vi "ASDE Signal Data Table For New_MS.vi"(4 "S Anal":T4, 6 "F ex Info":T3, 7 "S Table Z":T1, 8 "error in":errorcluster caption="エラー入力", 9 "S Table C2":T2={"R BL (pA)"=0.0, "R STD (pA)"=0.0, "U thre (pA)"=0.0, "D thre (pA)"=0.0, "U thre (n)"=0.0, "D thre (n)"=0.0, "STD smooth Point "=10, "MAX Duration time(s)"=0.01} {"MAX Duration time(s)" format="%#_13g"}, 10 "S Table C1":T6, 11 "S Table C0":T5) -> (0 "error out":errorcluster caption="エラー出力", 1 "S Peak Position Final (s)":dbl=1000.0 format="%#_13g", 2 "Signal R count (n)":i32, 3 "S Table Present Sum":string[][](table) caption="S Table Sum")   [LabVIEW 2018]
panel:
  out "S Table Tag X":string[](array[string])
  out "Signal Pre Count":i32
  out "LL Retention time":dbl
  out "S Peak Position Time (s) Pre":dbl=1000.0 format="%#_13g"
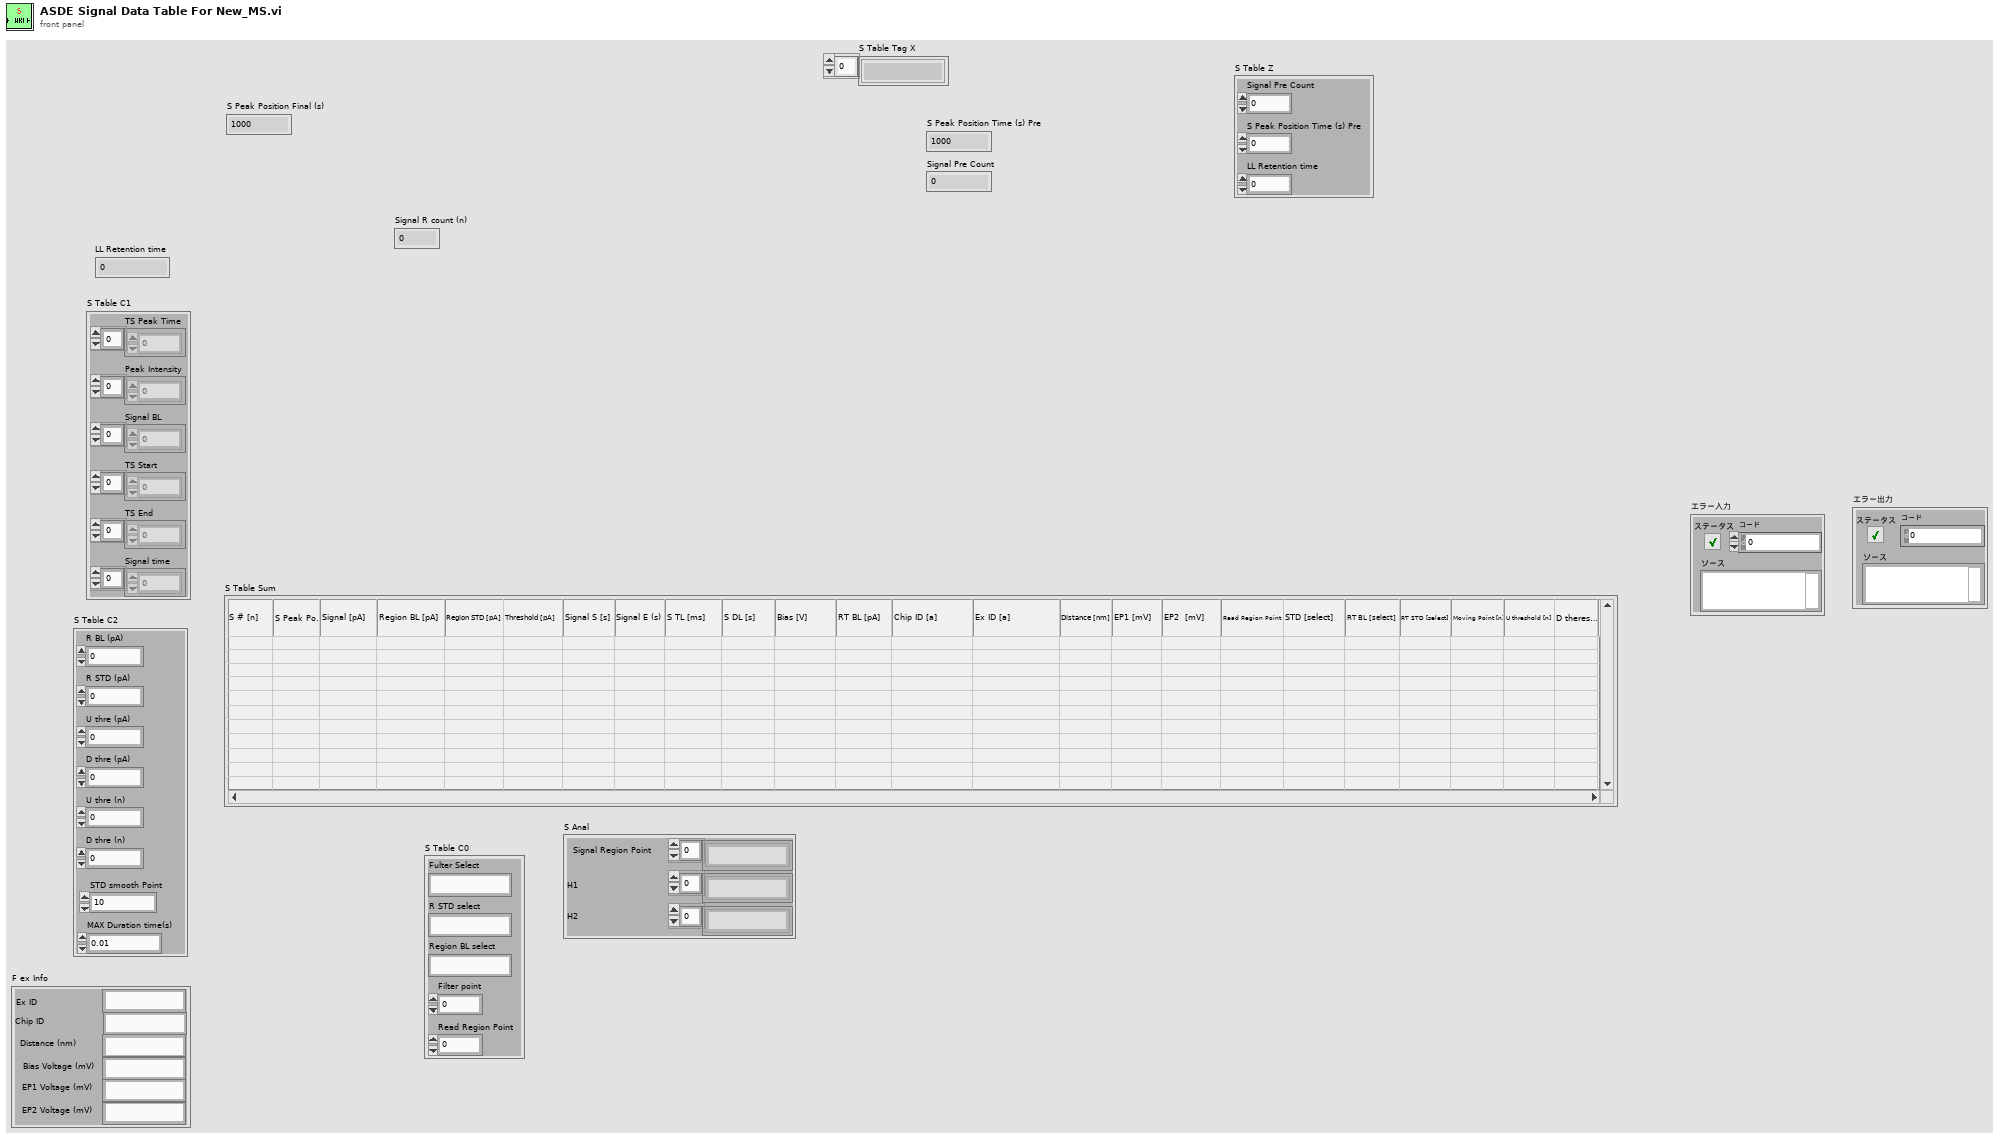
[diagram p1: front panel]
types:
  T1 = cluster{"Signal Pre Count":i32, "S Peak Position Time (s) Pre":dbl, "LL Retention time":dbl}
  T2 = cluster{"R BL (pA)":dbl, "R STD (pA)":dbl, "U thre (pA)":dbl, "D thre (pA)":dbl, "U thre (n)":dbl, "D thre (n)":dbl, "STD smooth Point ":i32, "MAX Duration time(s)":dbl}
  T3 = cluster{"Ex ID":string, "Chip ID":string, "Distance (nm)":string, "Bias Voltage (mV)":string, "EP1 Voltage (mV)":string, "EP2 Voltage (mV)":string}
  T4 = cluster{"Signal Region Point":string[], "H1":string[], "H2":string[]}
  T5 = cluster{"Fulter Select":string, "R STD select":string, "Region BL select":string, "Filter point":i32, "Read Region Point":i32}
  T6 = cluster{"TS Peak Time":dbl[], "Peak Intensity":dbl[], "Signal BL":dbl[], "TS Start":dbl[], "TS End":dbl[], "Signal time":dbl[]}
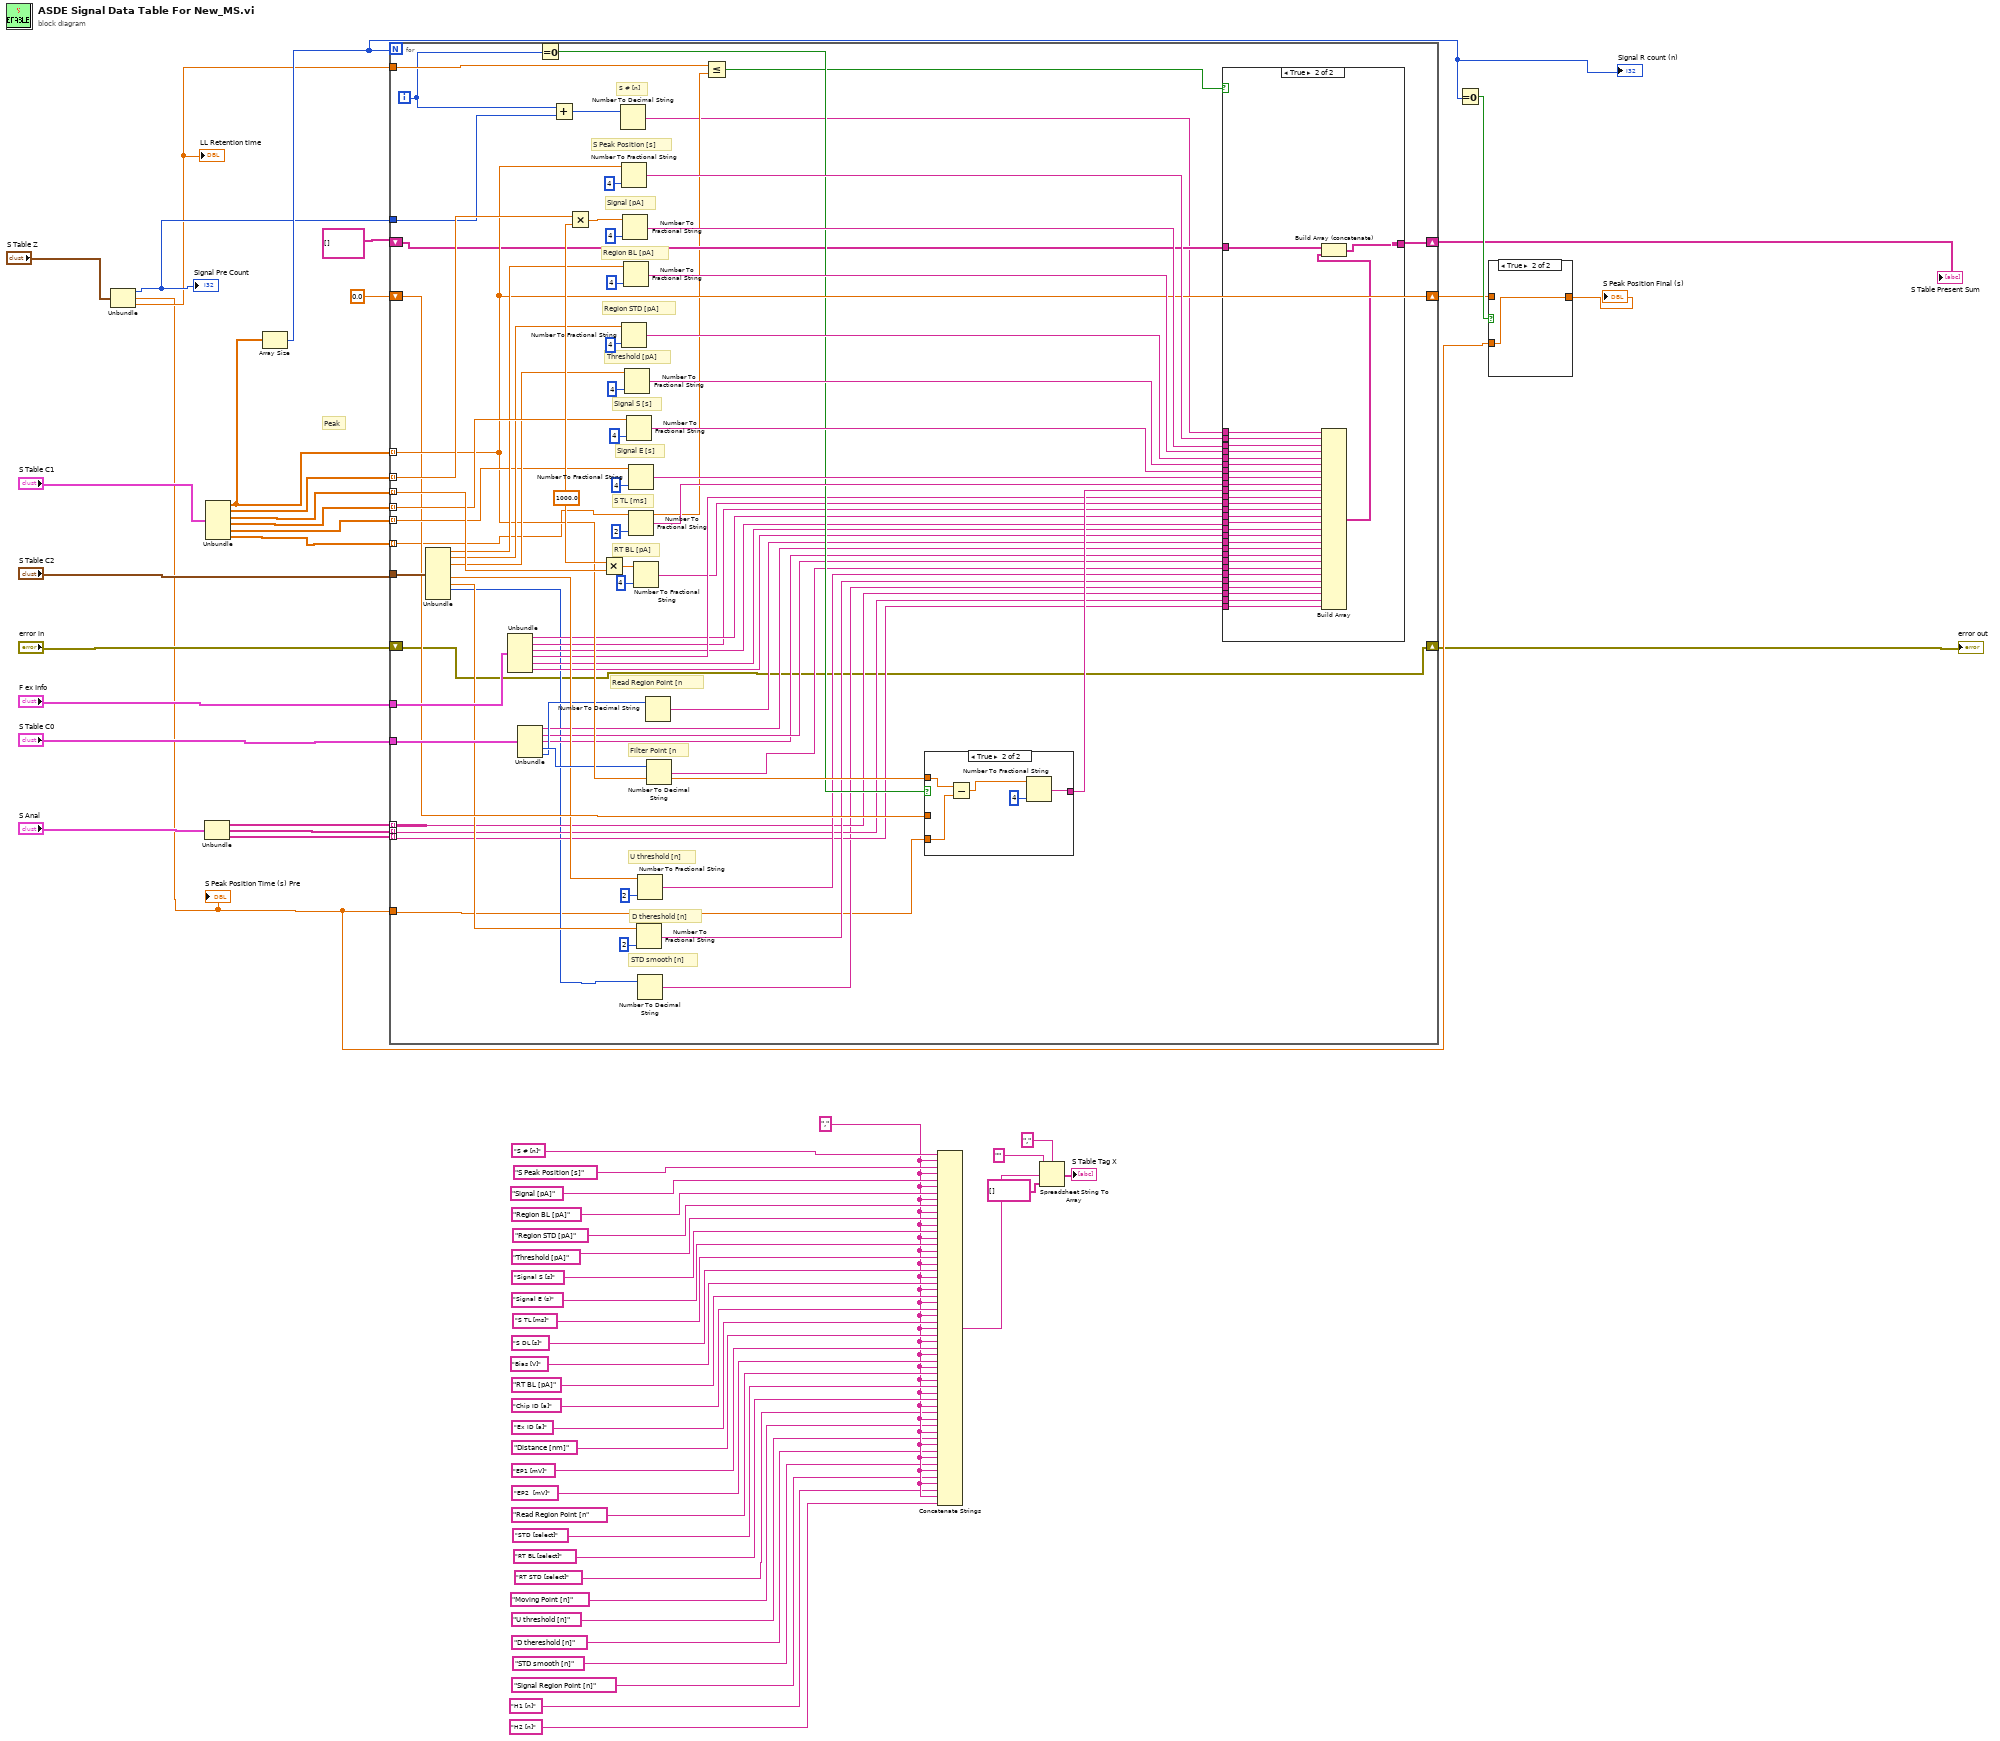
[diagram p0: block diagram]
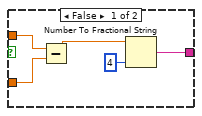
[diagram p4: hidden frame]
diagram:
  w20 = "," ("デリミタ（タブ）")
  # "Peak"
  n1 = Unbundle("S Table Z") -> ("Signal Pre Count"=w6:i32, "S Peak Position Time (s) Pre"=w4:dbl, "LL Retention time"=w5:dbl)
  "S Peak Position Time (s) Pre" <- w4
  "LL Retention time" <- w5
  "Signal Pre Count" <- w6
  n2 = Unbundle("S Anal") -> ("Signal Region Point"=w50:string[], "H1"=w49:string[], "H2"=w48:string[])
  n3 = Unbundle("S Table C1") -> ("TS Peak Time"=w60:dbl[], "Peak Intensity"=w59:dbl[], "Signal BL"=w58:dbl[], "TS Start"=w57:dbl[], "TS End"=w56:dbl[], "Signal time"=w55:dbl[])
  n4 = Array Size(array=w60) -> (size(s)=w8:i32)
  "Signal R count (n)" <- w8
  n5 = for {
    N: w8 -> [_]
    tunnel: w60 -> [w101] mode=indexing
    tunnel: w59 -> [w128] mode=indexing
    tunnel: "S Table C2" -> [w131]
    tunnel: "F ex Info" -> [w130]
    tunnel: w58 -> [w122] mode=indexing
    tunnel: w57 -> [w118] mode=indexing
    tunnel: w56 -> [w102] mode=indexing
    tunnel: w55 -> [w74] mode=indexing
    tunnel: "S Table C0" -> [w129]
    shift-right: [w101] -> w10
    shift-left: 0.0 -> [w100]
    shift-right: [w78] -> w2
    shift-left: string[][] [] -> [w77]
    tunnel: w5 -> [w75]
    tunnel: w50 -> [w73] mode=indexing
    tunnel: w49 -> [w72] mode=indexing
    tunnel: w48 -> [w71] mode=indexing
    tunnel: w6 -> [w68]
    tunnel: w4 -> [w63]
    shift-right: [w62] -> w1
    shift-left: "error in" -> [w62]
    i -> [w69]
    w120 = 1000.0 ("y")
    # "STD smooth [n]"
    # "D thereshold [n]"
    # "U threshold [n]"
    # "Filter Point [n"
    # "Read Region Point [n"
    # "RT BL [pA]"
    # "S TL [ms]"
    # "Signal E [s]"
    # "Signal S [s]"
    # "Threshold [pA]"
    # "Region STD [pA]"
    # "Region BL [pA]"
    # "Signal [pA]"
    # "S Peak Position [s]"
    # "S # [n]"
    n6 = Unbundle(w131) -> ("R BL (pA)"=w114:dbl, "R STD (pA)"=w110:dbl, "U thre (pA)"=w108:dbl, "U thre (n)"=w96:dbl, "D thre (n)"=w93:dbl, "STD smooth Point"=w65:i32)  [unwired: 2 out]
    n7 = Unbundle(w130) -> ("Ex ID"=w90:string, "Chip ID"=w89:string, "Distance (nm)"=w87:string, "Bias Voltage (mV)"=w91:string, "EP1 Voltage (mV)"=w92:string, "EP2 Voltage (mV)"=w70:string)
    n8 = Unbundle(w129) -> ("Fulter Select"=w80:string, "R STD select"=w82:string, "Region BL select"=w81:string, "Filter point"=w97:i32, "Read Region Point"=w86:i32)
    n9 = Equal To 0?(x=w69) -> (x = 0?=w98:bool)
    n10 = Add(x=w69, y=w68) -> (x+y=w67:i32)
    n11 = Multiply(x=w128, y=w120) -> (x*y=w126:dbl)
    n12 = Multiply(x=w120, y=w122) -> (x*y=w121:dbl)
    n13 = Number To Decimal String(number=w67) -> (decimal integer string=w66:string)  [unwired: 1 in]
    n14 = Number To Fractional String(number=w101, precision (6)=i16 4 ("精度（6）")) -> (F-format string=w127:string)  [unwired: 2 in]
    n15 = Number To Fractional String(number=w110, precision (6)=i16 4 ("精度（6）")) -> (F-format string=w109:string)  [unwired: 2 in]
    n16 = Number To Fractional String(number=w126, precision (6)=i16 4 ("精度（6）")) -> (F-format string=w125:string)  [unwired: 2 in]
    n17 = Number To Fractional String(number=w114, precision (6)=i16 4 ("精度（6）")) -> (F-format string=w112:string)  [unwired: 2 in]
    n18 = Number To Fractional String(number=w108, precision (6)=i16 4 ("精度（6）")) -> (F-format string=w106:string)  [unwired: 2 in]
    n19 = Number To Fractional String(number=w118, precision (6)=i16 4 ("精度（6）")) -> (F-format string=w105:string)  [unwired: 2 in]
    n20 = Number To Fractional String(number=w102, precision (6)=i16 4 ("精度（6）")) -> (F-format string=w104:string)  [unwired: 2 in]
    n21 = Number To Fractional String(number=w74, precision (6)=i16 2 ("精度（6）")) -> (F-format string=w103:string)  [unwired: 2 in]
    n22 = Number To Fractional String(number=w121, precision (6)=i16 4 ("精度（6）")) -> (F-format string=w88:string)  [unwired: 2 in]
    n23 = Number To Fractional String(number=w93, precision (6)=i16 2 ("精度（6）")) -> (F-format string=w85:string)  [unwired: 2 in]
    n24 = Number To Fractional String(number=w96, precision (6)=i16 2 ("精度（6）")) -> (F-format string=w84:string)  [unwired: 2 in]
    n25 = Number To Decimal String(number=w65) -> (decimal integer string=w64:string)  [unwired: 1 in]
    n26 = Number To Decimal String(number=w86) -> (decimal integer string=w79:string)  [unwired: 1 in]
    n27 = Number To Decimal String(number=w97) -> (decimal integer string=w83:string)  [unwired: 1 in]
    n28 = Less Or Equal?(x=w75, y=w74) -> (x <= y?=w76:bool)
    n29 = case shown="True" w98 {
      tunnel: w101 -> [w168 w169]
      tunnel: w100 -> [w167 _]
      tunnel: [w166 w173] -> w99
      tunnel: w63 -> [_ w170]
      frame False {
        n30 = Subtract(x=w168, y=w167) -> (x-y=w164:dbl)
        n31 = Number To Fractional String(number=w164, precision (6)=i16 4 ("精度（6）")) -> (F-format string=w166:string)  [unwired: 2 in]
      }
      frame True {
        n32 = Subtract(x=w169, y=w170) -> (x-y=w171:dbl)
        n33 = Number To Fractional String(number=w171, precision (6)=i16 4 ("精度（6）")) -> (F-format string=w173:string)  [unwired: 2 in]
      }
    }
    n34 = case shown="True" w76 {
      tunnel: w127 -> [_ w163]
      tunnel: w125 -> [_ w162]
      tunnel: w112 -> [_ w161]
      tunnel: w109 -> [_ w160]
      tunnel: w106 -> [_ w159]
      tunnel: w105 -> [_ w158]
      tunnel: w104 -> [_ w157]
      tunnel: w103 -> [_ w156]
      tunnel: w99 -> [_ w155]
      tunnel: w92 -> [_ w154]
      tunnel: w91 -> [_ w153]
      tunnel: w90 -> [_ w152]
      tunnel: w89 -> [_ w151]
      tunnel: w88 -> [_ w150]
      tunnel: w87 -> [_ w149]
      tunnel: w64 -> [_ w134]
      tunnel: w85 -> [_ w138]
      tunnel: w84 -> [_ w139]
      tunnel: w83 -> [_ w140]
      tunnel: w82 -> [_ w141]
      tunnel: w81 -> [_ w142]
      tunnel: w80 -> [_ w143]
      tunnel: w79 -> [_ w144]
      tunnel: [w132 w147] -> w78
      tunnel: w77 -> [w132 w146]
      tunnel: w73 -> [_ w135]
      tunnel: w72 -> [_ w136]
      tunnel: w71 -> [_ w137]
      tunnel: w70 -> [_ w145]
      tunnel: w66 -> [_ w133]
      frame False {
      }
      frame True {
        n35 = Build Array(w133, w163, w162, w161, w160, w159, w158, w157, w156, w155, w153, w150, w151, w152, w149, w154, w145, w144, w143, w142, w141, w140, w139, w138, w134, w135, w136, w137) -> (w148:string[])
        n36 = Build Array (concatenate)(w146, w148) -> (w147:string[][])
      }
    }
  }
  "S Table Present Sum" <- w2
  "error out" <- w1
  n37 = Concatenate Strings("S # [n]" ("文字列"), w20, "S Peak Position [s]" ("文字列"), w20, "Signal [pA]" ("文字列"), w20, "Region BL [pA]" ("文字列"), w20, "Region STD [pA]" ("文字列"), w20, "Threshold [pA]" ("文字列"), w20, "Signal S [s]" ("文字列"), w20, "Signal E (s)" ("文字列"), w20, "S TL [ms]" ("文字列"), w20, "S DL [s]" ("文字列"), w20, "Bias [V]" ("文字列"), w20, "RT BL [pA]" ("文字列"), w20, "Chip ID [a]" ("文字列"), w20, "Ex ID [a]" ("文字列"), w20, "Distance [nm]" ("文字列"), w20, "EP1 [mV]" ("文字列"), w20, "EP2  [mV]" ("文字列"), w20, "Read Region Point [n" ("文字列"), w20, "STD [select]" ("文字列"), w20, "RT BL [select]" ("文字列"), w20, "RT STD [select]" ("文字列"), w20, "Moving Point [n]" ("文字列"), w20, "U threshold [n]" ("文字列"), w20, "D thereshold [n]" ("文字列"), w20, "STD smooth [n]" ("文字列"), w20, "Signal Region Point [n]" ("文字列"), w20, "H1 [n]" ("文字列"), w20, "H2 [n]" ("文字列")) -> (w42:string)
  n38 = Spreadsheet String To Array(delimiter (Tab)="," ("デリミタ（タブ）"), format string="" ("形式文字列"), spreadsheet string=w42, array type (2D Dbl)=string[] [] ("行ヘッダ文字列[]")) -> (array=→"S Table Tag X":string[])
  n39 = Equal To 0?(x=w8) -> (x = 0?=w11:bool)
  n40 = case shown="True" w11 {
    tunnel: w10 -> [w174 _]
    tunnel: [w174 w175] -> w7
    tunnel: w4 -> [_ w175]
    frame False {
    }
    frame True {
    }
  }
  "S Peak Position Final (s)" <- w7
